vi "List.vi"(8 "error in (no error)":errorcluster) -> (0 "error out":errorcluster, 3 "registered loggers":string[](array[string]))   [LabVIEW 2018, in "GLog.lvlib" / "Registry.lvlib"]
uses:
  Registry.lvlib
  Registry Actions.ctl
  dependencies/Utilities/Utilities.lvlib
panel:
  # "Connector Pane"
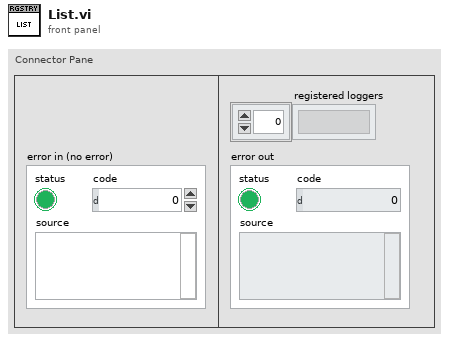
[diagram p1: front panel]
types:
  T1 = typedef "GLog.lvlib/Registry.lvlib/Registry Actions.ctl" = enum16{"Register", "Log", "Enable", "Enable All", "Disable", "Disable All", "Get Enable State", "Get Minimum Log Level", "Set Minimum Log Level", "Set All Minimum Log Level", "Get Logger Info", "Get All Logger Info", "List", "Unregister", "Unregister All", "Shutdown"}
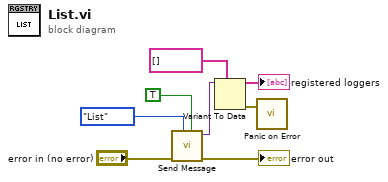
[diagram p0: block diagram]
diagram:
  n1 = call "Send Message.vi"("return data? (F)"=TRUE ("return data?"), "action"=Registry_Actions."List", "error in (no error)"="error in (no error)") -> ("error out"=→"error out":errorcluster, "Variant"=w6:variant)  [unwired: 7 in]
  n2 = Variant To Data(type=string[] [], Variant=w6) -> (data=→"registered loggers":string[], error out=w4:errorcluster)  [unwired: 1 in]
  n3 = call "Panic on Error.vi"("error in (no error)"=w4) -> ()  [unwired: 3 in]
